vi "RemoteVI Cursor Outside Window.vi"(0 "hWnd":u64) -> (4 "outside?":bool)   [LabVIEW 2020, in "RemoteVI.lvlib"]
doc: "TRUE when the host cursor (user32 GetCursorPos) lies outside the window rectangle of hWnd (user32 GetWindowRect, right and bottom exclusive). FALSE when either call fails. Used by the server loop to tell a tip strip that can only stem from the remote pointer. No VI Server call."
uses:
  RemoteVI.lvlib
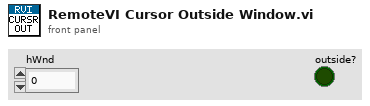
[diagram p1: front panel]
types:
  T1 = cluster{"left":i32, "top":i32, "right":i32, "bottom":i32}
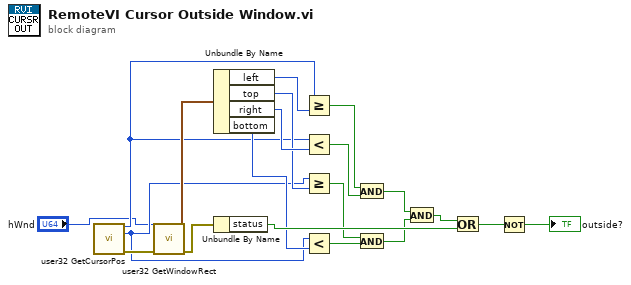
[diagram p0: block diagram]
diagram:
  n1 = call "user32 GetCursorPos.vi"() -> ("X"=w2:i32, "Y"=w3:i32, "error out"=w4:errorcluster)  [unwired: 12 in, 1 out]
  n2 = call "user32 GetWindowRect.vi"("hWnd"="hWnd", "error in"=w4) -> ("RECT"=w5:T1, "error out"=w6:errorcluster)  [unwired: 11 in, 1 out]
  n3 = Unbundle By Name(w5) -> ("left"=w7:i32, "top"=w8:i32, "right"=w9:i32, "bottom"=w10:i32)
  n4 = Unbundle By Name(w6) -> ("status"=w18:bool)
  n5 = Greater Or Equal?(x=w2, y=w7) -> (x >= y?=w11:bool)
  n6 = Less?(x=w2, y=w9) -> (x < y?=w12:bool)
  n7 = Greater Or Equal?(x=w3, y=w8) -> (x >= y?=w13:bool)
  n8 = Less?(x=w3, y=w10) -> (x < y?=w14:bool)
  n9 = And(x=w11, y=w12) -> (x .and. y?=w15:bool)
  n10 = And(x=w13, y=w14) -> (x .and. y?=w16:bool)
  n11 = And(x=w15, y=w16) -> (x .and. y?=w17:bool)
  n12 = Or(x=w17, y=w18) -> (x .or. y?=w19:bool)
  n13 = Not(x=w19) -> (.not. x?=→"outside?":bool)
